vi "Test Buffer Preview.vi"() -> (0 "error out":errorcluster)   [LabVIEW 2026]
doc: "HAL-BUF-001: reading buffered data previews exact data without consuming the queue."
uses:
  source/framework/Hardware/Hardware.lvclass
  source/framework/Hardware/Hardware.lvclass/Hardware.ctl
  <vilib>/addons/_JKI Toolkits/Caraya/classes/Test/Test.lvclass
  <vilib>/addons/_JKI Toolkits/Caraya/classes/Assert/Assert.lvclass
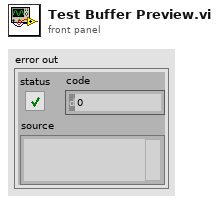
[diagram p1: front panel]
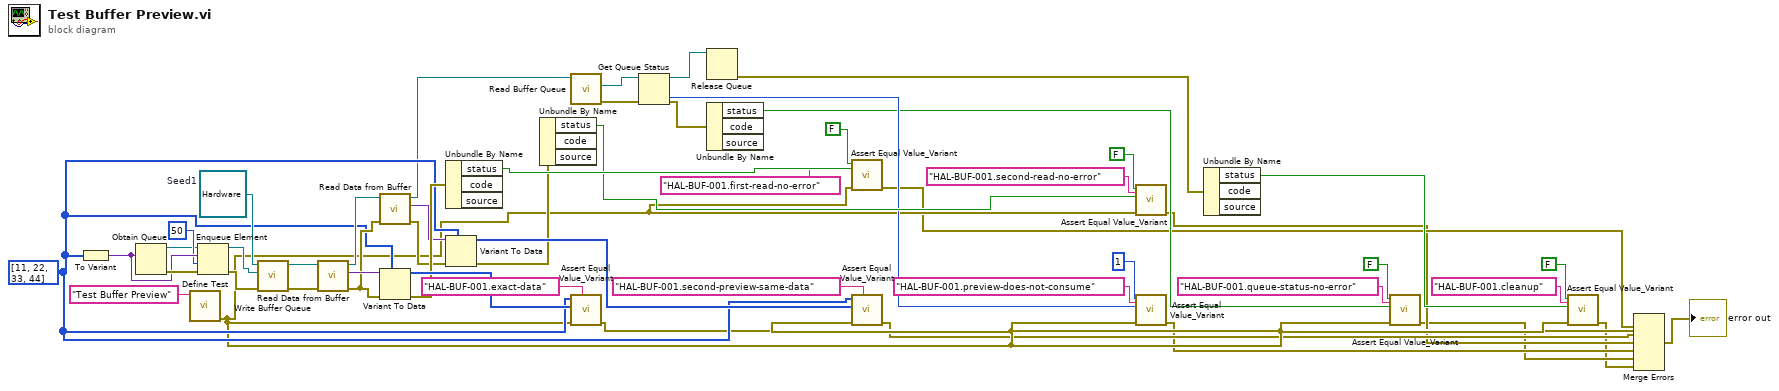
[diagram p0: block diagram]
diagram:
  w29 = i32[] [11, 22, 33, 44]
  w46 = refnum<class "Hardware.lvclass"> refnum  # Seed1
  n1 = To Variant(anything=w29) -> (Variant=w50:variant)
  n2 = Obtain Queue(element data type=w50) -> (queue out=w48:refnum<queue>, error out=w51:errorcluster)  [unwired: 4 in, 1 out]
  n3 = call <vilib>:"Define Test.vi"("Label (VI Title)"="Test Buffer Preview") -> ("error out"=w11:errorcluster)  [unwired: 9 in, 1 out]
  n4 = Enqueue Element(queue=w48, element=w50, timeout in ms (-1)=50, error in (no error)=w51) -> (queue out=w45:refnum<queue>, error out=w47:errorcluster)  [unwired: 1 out]
  n5 = call "Write Buffer Queue.vi"("error in (no error)"=w47, "Buffer Queue"=w45, "Hardware in"=w46) -> ("error out"=w44:errorcluster, "Hardware out"=w43:refnum<class "Hardware.lvclass">)  [unwired: 7 in]
  n6 = call "Read Data from Buffer.vi"("error in (no error)"=w44, "Hardware in"=w43) -> ("error out"=w35:errorcluster, "Variant"=w42:variant, "Hardware out"=w34:refnum<class "Hardware.lvclass">)  [unwired: 7 in]
  n7 = call "Read Data from Buffer.vi"("error in (no error)"=w35, "Hardware in"=w34) -> ("error out"=w32:errorcluster, "Variant"=w33:variant, "Hardware out"=w24:refnum<class "Hardware.lvclass">)  [unwired: 7 in]
  n8 = Variant To Data(error in=w35, type=w29, Variant=w42) -> (data=w41:i32[], error out=w39:errorcluster)
  n9 = Unbundle By Name(w39) -> ("status"=w38:bool)  [unwired: 2 out]
  n10 = Variant To Data(error in=w32, type=w29, Variant=w33) -> (data=w31:i32[], error out=w28:errorcluster)
  n11 = Unbundle By Name(w28) -> ("status"=w27:bool)  [unwired: 2 out]
  n12 = call "Read Buffer Queue.vi"("Hardware in"=w24) -> ("error out"=w23:errorcluster, "Buffer Queue"=w22:refnum<queue>)  [unwired: 8 in, 1 out]
  n13 = call <vilib>:"Assert Equal Value_Variant.vi"("Label"="HAL-BUF-001.exact-data", "error in (no error)"=w11, "Actual"=w41, "Expected"=w29) -> ("error out"=w8:errorcluster)  [unwired: 6 in, 1 out]
  n14 = Get Queue Status(queue=w22, error in (no error)=w23) -> (queue out=w14:refnum<queue>, error out=w18:errorcluster, # elements in queue=w21:i32)  [unwired: 1 in, 5 out]
  n15 = Release Queue(queue=w14) -> (error out=w13:errorcluster)  [unwired: 2 in, 2 out]
  n16 = Unbundle By Name(w18) -> ("status"=w17:bool)  [unwired: 2 out]
  n17 = call <vilib>:"Assert Equal Value_Variant.vi"("Label"="HAL-BUF-001.first-read-no-error", "error in (no error)"=w11, "Actual"=w38, "Expected"=FALSE) -> ("error out"=w7:errorcluster)  [unwired: 6 in, 1 out]
  n18 = call <vilib>:"Assert Equal Value_Variant.vi"("Label"="HAL-BUF-001.second-preview-same-data", "error in (no error)"=w11, "Actual"=w31, "Expected"=w29) -> ("error out"=w6:errorcluster)  [unwired: 6 in, 1 out]
  n19 = call <vilib>:"Assert Equal Value_Variant.vi"("Label"="HAL-BUF-001.second-read-no-error", "error in (no error)"=w11, "Actual"=w27, "Expected"=FALSE) -> ("error out"=w5:errorcluster)  [unwired: 6 in, 1 out]
  n20 = call <vilib>:"Assert Equal Value_Variant.vi"("Label"="HAL-BUF-001.preview-does-not-consume", "error in (no error)"=w11, "Actual"=w21, "Expected"=1) -> ("error out"=w4:errorcluster)  [unwired: 6 in, 1 out]
  n21 = Unbundle By Name(w13) -> ("status"=w12:bool)  [unwired: 2 out]
  n22 = call <vilib>:"Assert Equal Value_Variant.vi"("Label"="HAL-BUF-001.queue-status-no-error", "error in (no error)"=w11, "Actual"=w17, "Expected"=FALSE) -> ("error out"=w3:errorcluster)  [unwired: 6 in, 1 out]
  n23 = call <vilib>:"Assert Equal Value_Variant.vi"("Label"="HAL-BUF-001.cleanup", "error in (no error)"=w11, "Actual"=w12, "Expected"=FALSE) -> ("error out"=w2:errorcluster)  [unwired: 6 in, 1 out]
  n24 = Merge Errors(w8, w7, w6, w5, w4, w3, w2) -> (→"error out":errorcluster)
